vi "Logs.vi"(10 "字符串":string, 11 "Data Cluster":T1) -> (3 "Module Data":T1)   [LabVIEW 2025, in "Auto-Process.lvlib"]
uses:
  Auto-Process.lvlib
  Module Data--cluster.ctl
  Database/Database_access.lvclass
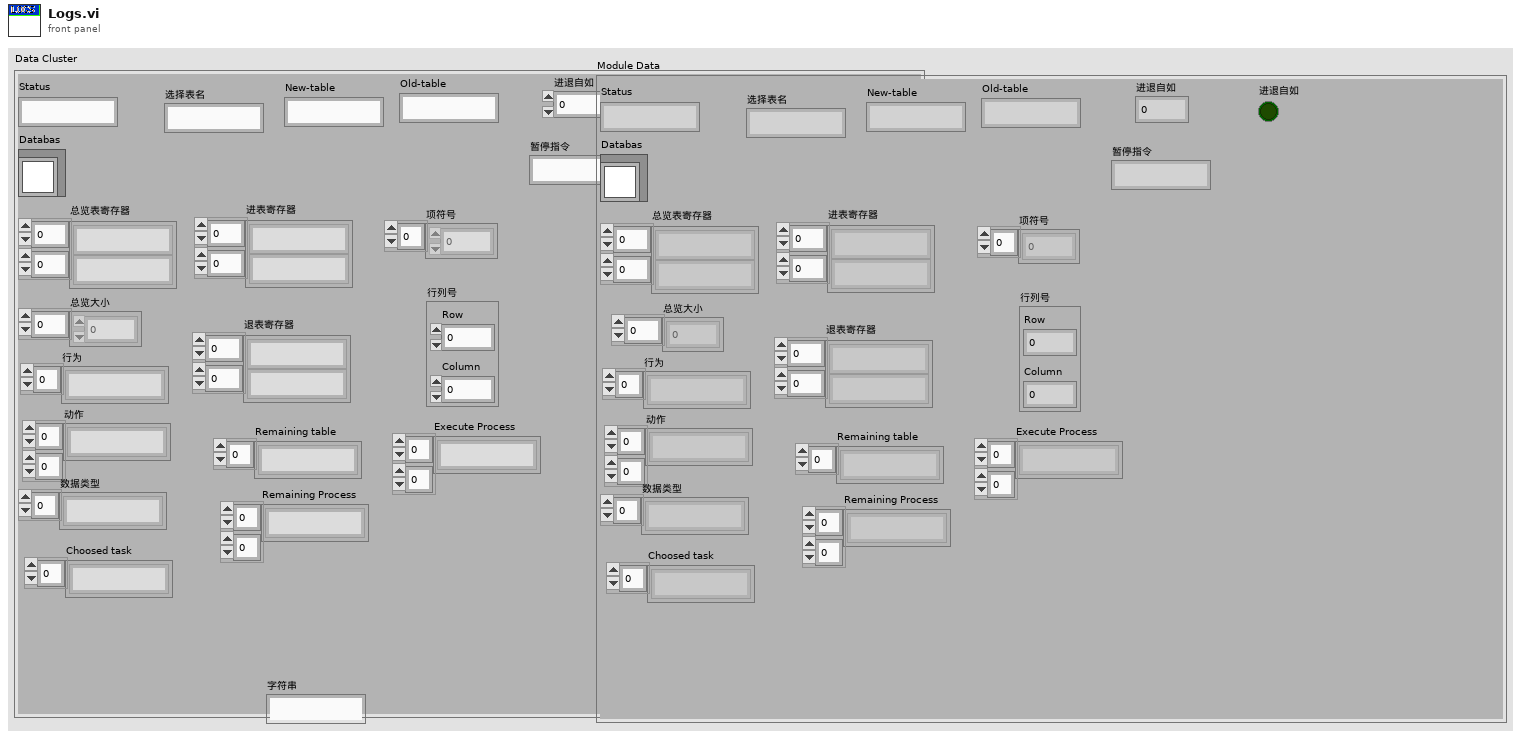
[diagram p1: front panel]
types:
  T1 = typedef "Auto-Process.lvlib/Module Data--cluster.ctl" = cluster{"Status":string, "Databas":refnum<class "Database_access.lvclass">, "总览表寄存器":string[][], "总览大小":i32[], "动作":string[][], "行为":string[], "数据类型":string[], "进表寄存器":string[][], "退表寄存器":string[][], "进退自如":u8, "选择表名":string, "New-table":string, "Old-table":string, "进退自如":bool, "行列号":cluster{"Row":i32, "Column":i32}, "项符号":i32[], "Choosed task":string[], "Remaining table":string[], "Remaining Process":string[][], "Execute Process":string[][], "暂停指令":string}
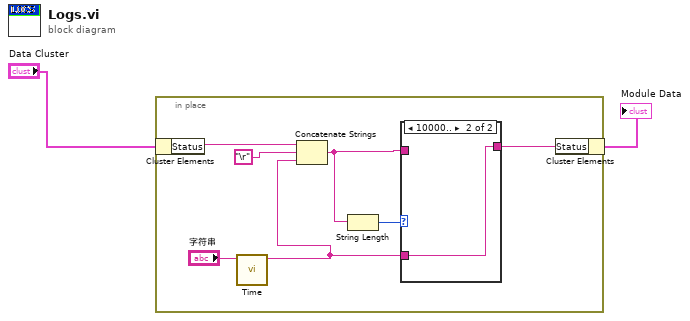
[diagram p0: block diagram]
diagram:
  n1 = in-place {
    n2 = in-place-cluster #1("Data Cluster") -> ("Status"=w9:string)
    n3 = call "Time.vi"("字符串"="字符串") -> ("连接的字符串"=w3:string)  [unwired: 10 in]
    n4 = Concatenate Strings(w9, "\r", w3) -> (w5:string)
    n5 = String Length(string=w5) -> (length=w6:i32)
    n6 = case shown="10000.." w6 {
      tunnel: w5 -> [w10 _]
      tunnel: [w10 w11] -> w4
      tunnel: w3 -> [_ w11]
      frame 0, Default {
      }
      frame 10000.. {
      }
    }
    n7 = in-place-cluster #1("Status"=w4) -> (→"Module Data":T1)
  }
